vi "single-point-cal.vi"(8 "TC5:8 Zero Point Offset":T1, 9 "TC1:4 Zero point offset":T2, 11 "adam5000:all-data-in":T3) -> (3 "adam5000:all-data-out":T3)   [LabVIEW 2024]
uses:
  controls/thermocouple-input-cluster.ctl
  controls/analog-input-cluster.ctl
  controls/analog-output-cluster.ctl
  controls/digitial-input-cluster.ctl
  controls/digital-output-cluster.ctl
  controls/adam-5000-all-module-datas.ctl
  controls/adam-5000-all-chassis-data.ctl
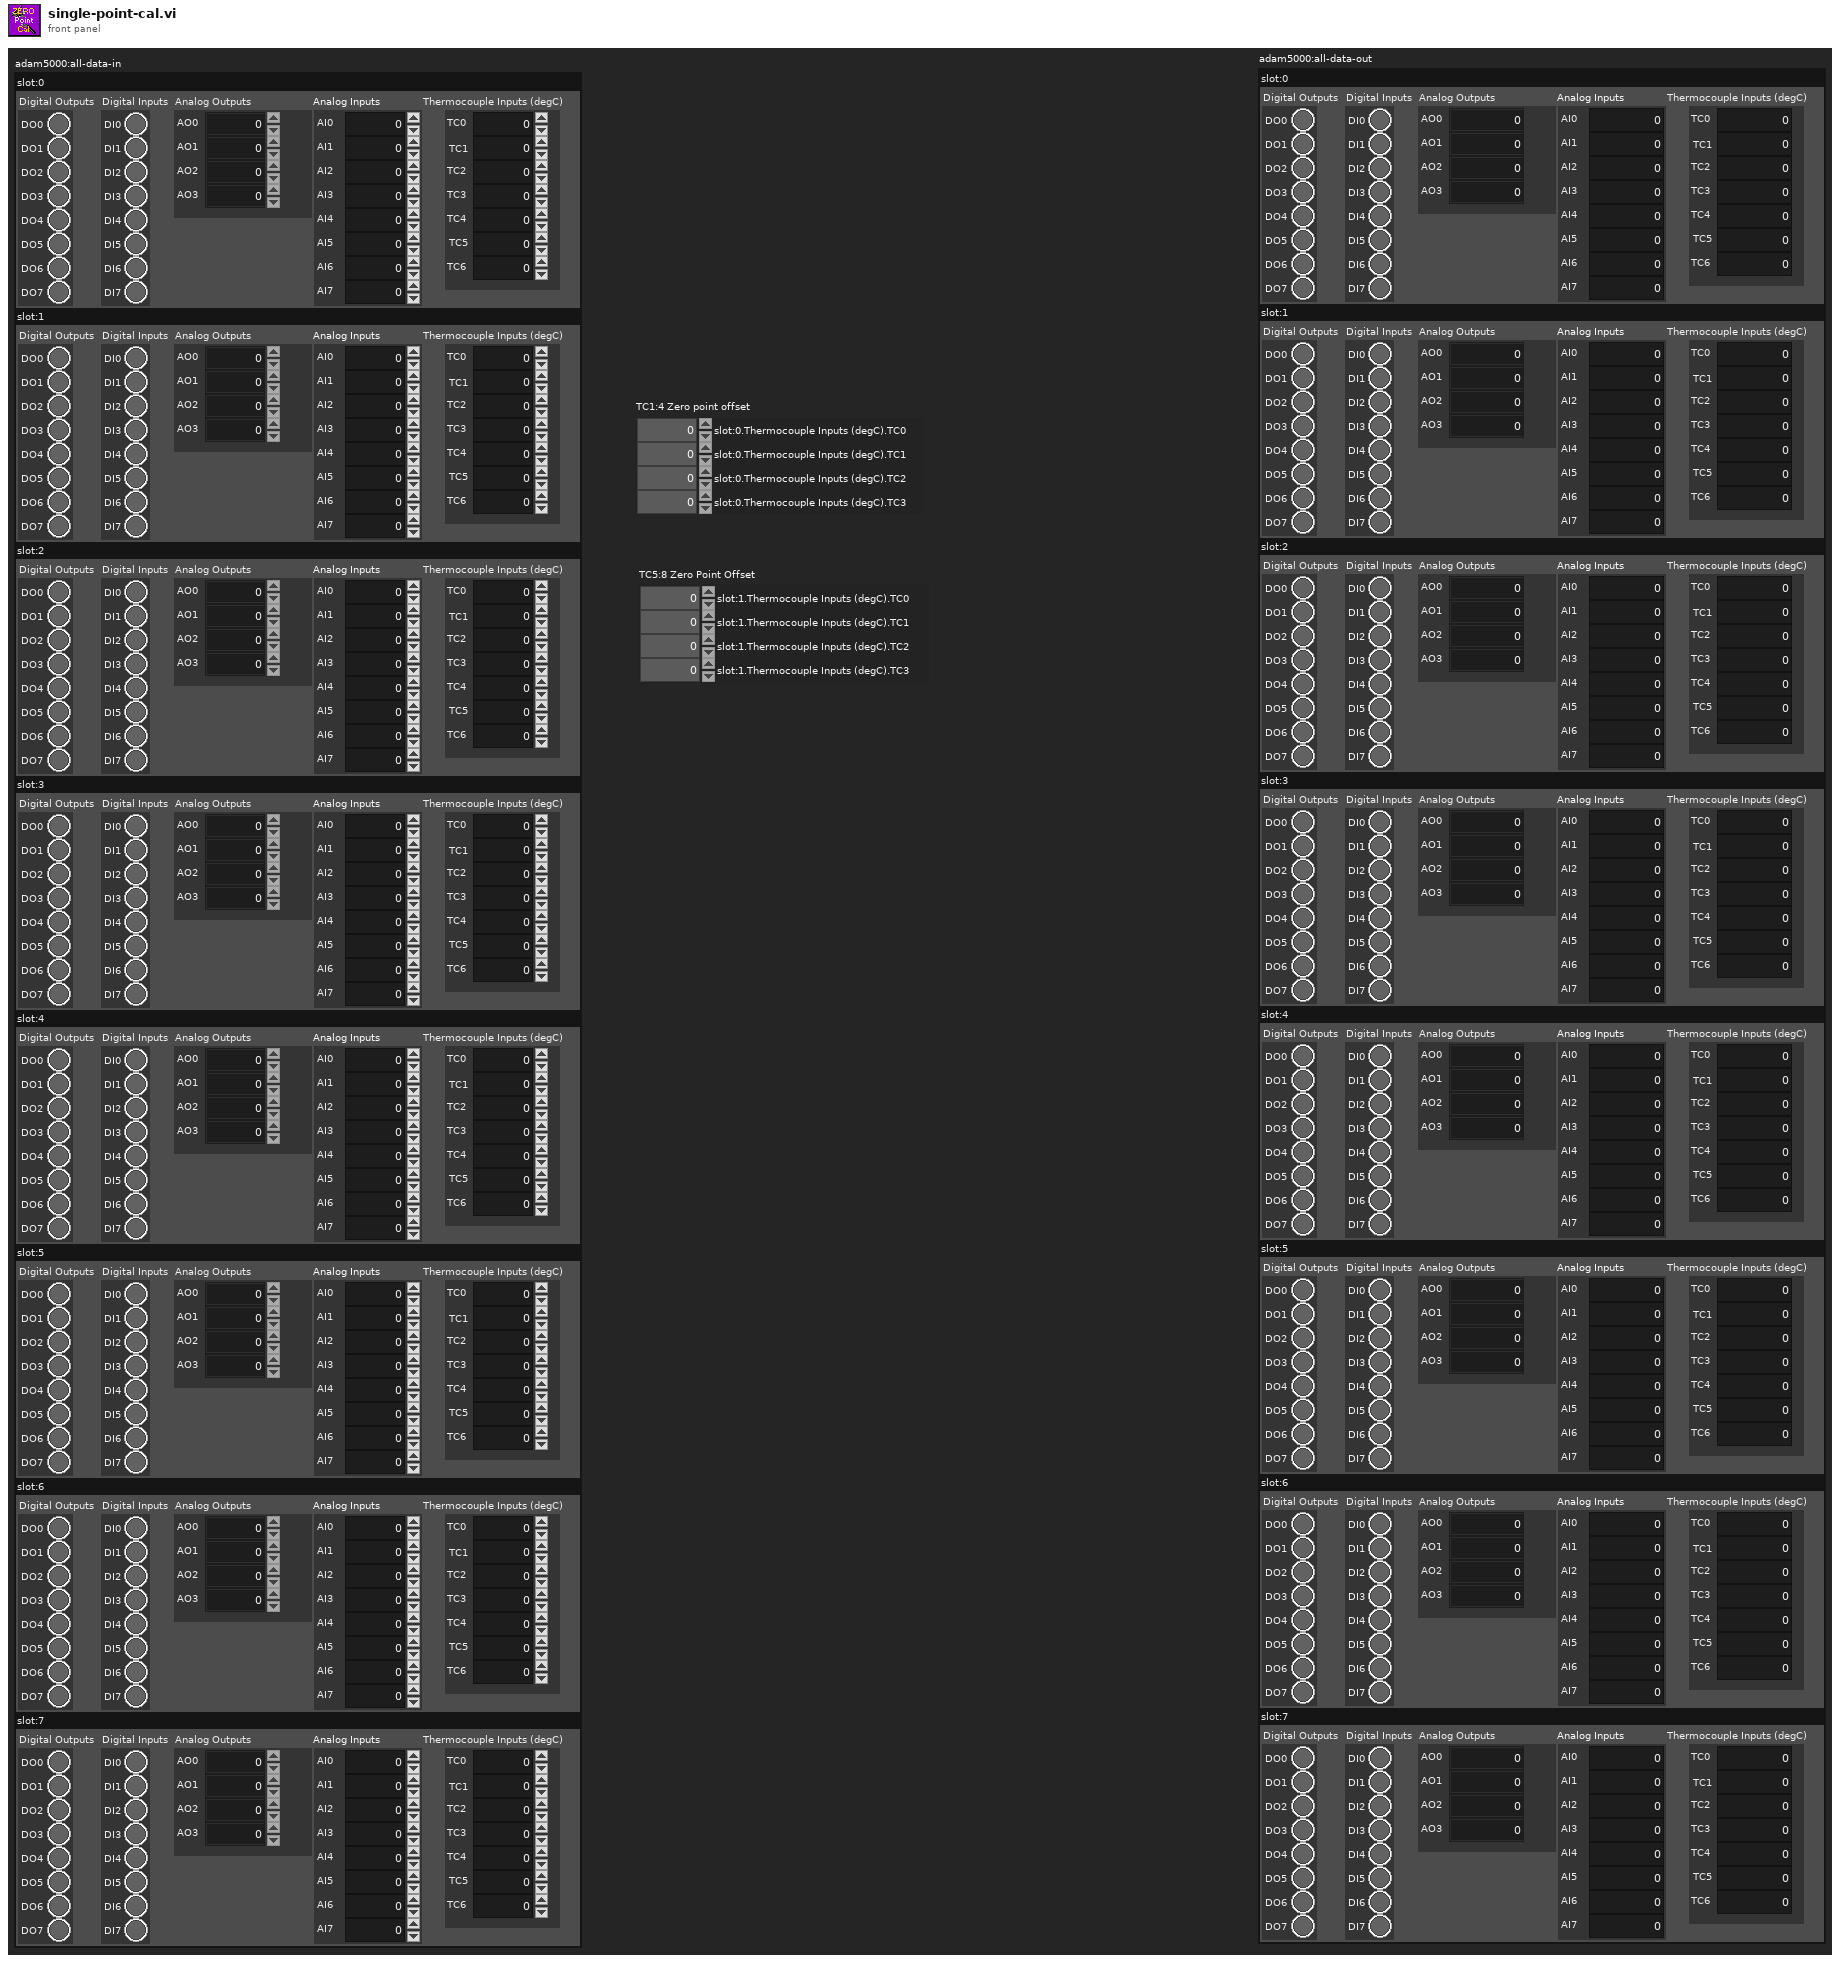
[diagram p1: front panel]
types:
  T1 = cluster{"slot:1.Thermocouple Inputs (degC).TC0":dbl, "slot:1.Thermocouple Inputs (degC).TC1":dbl, "slot:1.Thermocouple Inputs (degC).TC2":dbl, "slot:1.Thermocouple Inputs (degC).TC3":dbl}
  T2 = cluster{"slot:0.Thermocouple Inputs (degC).TC0":dbl, "slot:0.Thermocouple Inputs (degC).TC1":dbl, "slot:0.Thermocouple Inputs (degC).TC2":dbl, "slot:0.Thermocouple Inputs (degC).TC3":dbl}
  T3 = typedef "adam-5000-all-chassis-data.ctl" = cluster{"slot:0":T4, "slot:1":T4, "slot:2":T4, "slot:3":T4, "slot:4":T4, "slot:5":T4, "slot:6":T4, "slot:7":T4}
  T4 = typedef "adam-5000-all-module-datas.ctl" = cluster{"Digital Outputs":T5, "Digital Inputs":T6, "Analog Outputs":T7, "Analog Inputs":T8, "Thermocouple Inputs (degC)":T9}
  T5 = typedef "digital-output-cluster.ctl" = cluster{"DO0":bool, "DO1":bool, "DO2":bool, "DO3":bool, "DO4":bool, "DO5":bool, "DO6":bool, "DO7":bool}
  T6 = typedef "digitial-input-cluster.ctl" = cluster{"DI0":bool, "DI1":bool, "DI2":bool, "DI3":bool, "DI4":bool, "DI5":bool, "DI6":bool, "DI7":bool}
  T7 = typedef "analog-output-cluster.ctl" = cluster{"AO0":dbl, "AO1":dbl, "AO2":dbl, "AO3":dbl}
  T8 = typedef "analog-input-cluster.ctl" = cluster{"AI0":dbl, "AI1":dbl, "AI2":dbl, "AI3":dbl, "AI4":dbl, "AI5":dbl, "AI6":dbl, "AI7":dbl}
  T9 = typedef "thermocouple-input-cluster.ctl" = cluster{"TC0":dbl, "TC1":dbl, "TC2":dbl, "TC3":dbl, "TC4":dbl, "TC5":dbl, "TC6":dbl}
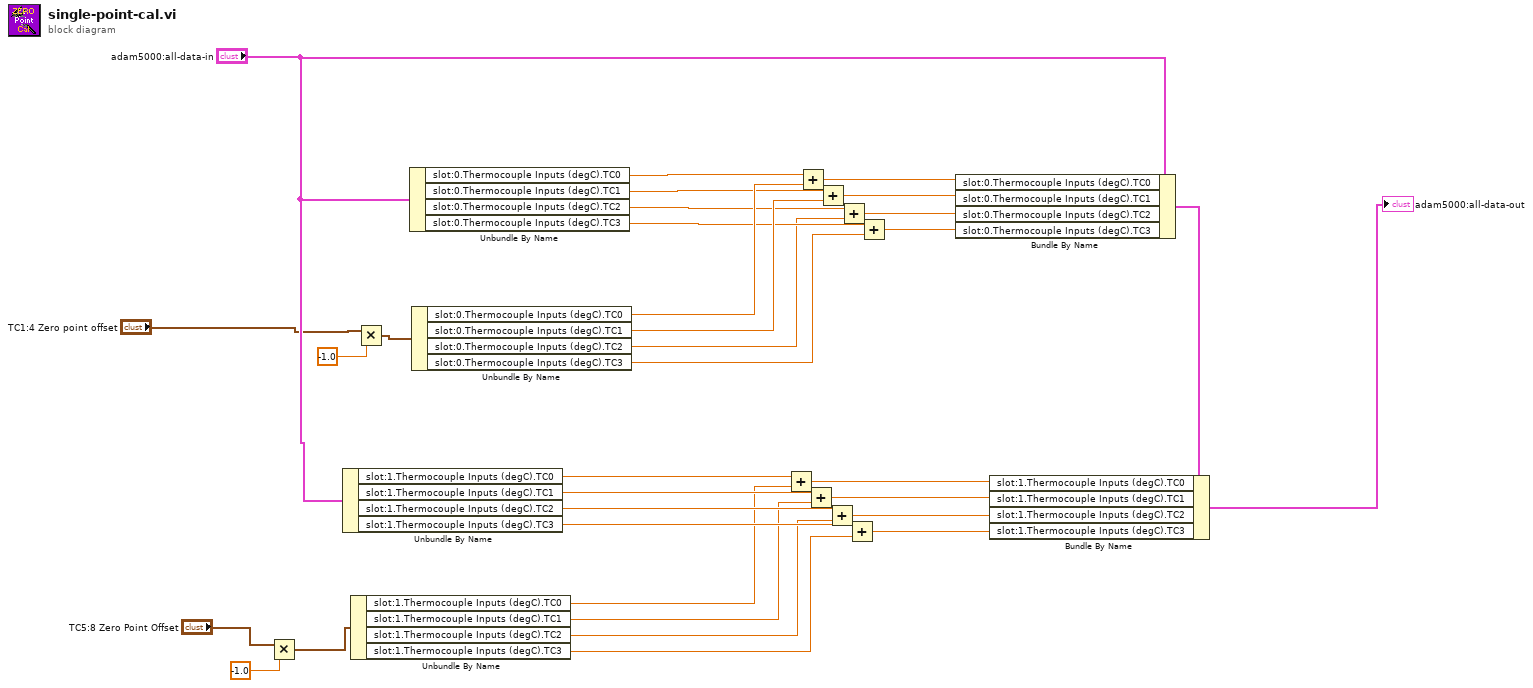
[diagram p0: block diagram]
diagram:
  n1 = Multiply(x="TC5:8 Zero Point Offset", y=-1.0) -> (x*y=w26:T1)
  n2 = Unbundle By Name("adam5000:all-data-in") -> ("slot:1.Thermocouple Inputs (degC).TC0"=w12:dbl, "slot:1.Thermocouple Inputs (degC).TC1"=w11:dbl, "slot:1.Thermocouple Inputs (degC).TC2"=w10:dbl, "slot:1.Thermocouple Inputs (degC).TC3"=w9:dbl)
  n3 = Unbundle By Name(w26) -> ("slot:1.Thermocouple Inputs (degC).TC0"=w8:dbl, "slot:1.Thermocouple Inputs (degC).TC1"=w7:dbl, "slot:1.Thermocouple Inputs (degC).TC2"=w6:dbl, "slot:1.Thermocouple Inputs (degC).TC3"=w5:dbl)
  n4 = Multiply(x="TC1:4 Zero point offset", y=-1.0) -> (x*y=w29:T2)
  n5 = Unbundle By Name("adam5000:all-data-in") -> ("slot:0.Thermocouple Inputs (degC).TC0"=w33:dbl, "slot:0.Thermocouple Inputs (degC).TC1"=w24:dbl, "slot:0.Thermocouple Inputs (degC).TC2"=w22:dbl, "slot:0.Thermocouple Inputs (degC).TC3"=w21:dbl)
  n6 = Unbundle By Name(w29) -> ("slot:0.Thermocouple Inputs (degC).TC0"=w25:dbl, "slot:0.Thermocouple Inputs (degC).TC1"=w23:dbl, "slot:0.Thermocouple Inputs (degC).TC2"=w20:dbl, "slot:0.Thermocouple Inputs (degC).TC3"=w19:dbl)
  n7 = Add(x=w12, y=w8) -> (x+y=w1:dbl)
  n8 = Add(x=w33, y=w25) -> (x+y=w17:dbl)
  n9 = Add(x=w11, y=w7) -> (x+y=w2:dbl)
  n10 = Add(x=w24, y=w23) -> (x+y=w16:dbl)
  n11 = Add(x=w10, y=w6) -> (x+y=w3:dbl)
  n12 = Add(x=w22, y=w20) -> (x+y=w15:dbl)
  n13 = Add(x=w9, y=w5) -> (x+y=w4:dbl)
  n14 = Add(x=w21, y=w19) -> (x+y=w14:dbl)
  n15 = Bundle By Name(cluster="adam5000:all-data-in", "slot:0.Thermocouple Inputs (degC).TC0"=w17, "slot:0.Thermocouple Inputs (degC).TC1"=w16, "slot:0.Thermocouple Inputs (degC).TC2"=w15, "slot:0.Thermocouple Inputs (degC).TC3"=w14) -> (w18:T3)
  n16 = Bundle By Name(cluster=w18, "slot:1.Thermocouple Inputs (degC).TC0"=w1, "slot:1.Thermocouple Inputs (degC).TC1"=w2, "slot:1.Thermocouple Inputs (degC).TC2"=w3, "slot:1.Thermocouple Inputs (degC).TC3"=w4) -> (→"adam5000:all-data-out":T3)
